vi "NR do Call Process.vi"(8 "error in (no error)":errorcluster caption="에러 입력(에러 없음)", 9 "Waiting Time":i32, 10 "Max Retry Count":i32, 11 "Instrument Manager 입력":refnum<class "Instrument Manager.lvclass">) -> (0 "error out":errorcluster caption="에러 출력", 2 "Connected?":bool, 3 "Instrument Manager 출력":refnum<class "Instrument Manager.lvclass">)   [LabVIEW 2023, in "Instrument Manager.lvclass"]
uses:
  Instrument Manager.lvclass
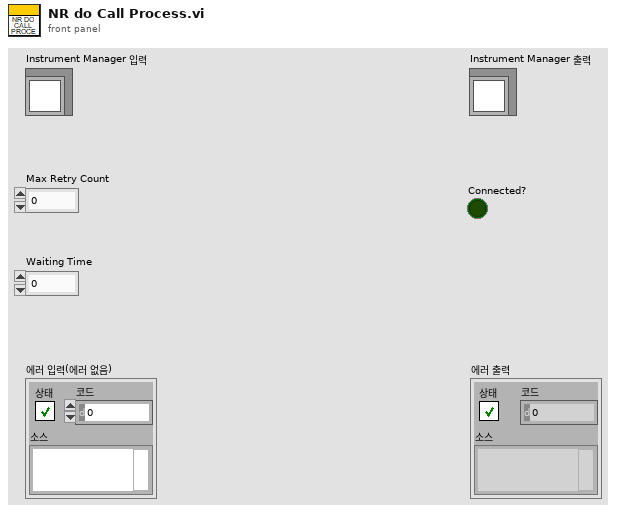
[diagram p1: front panel]
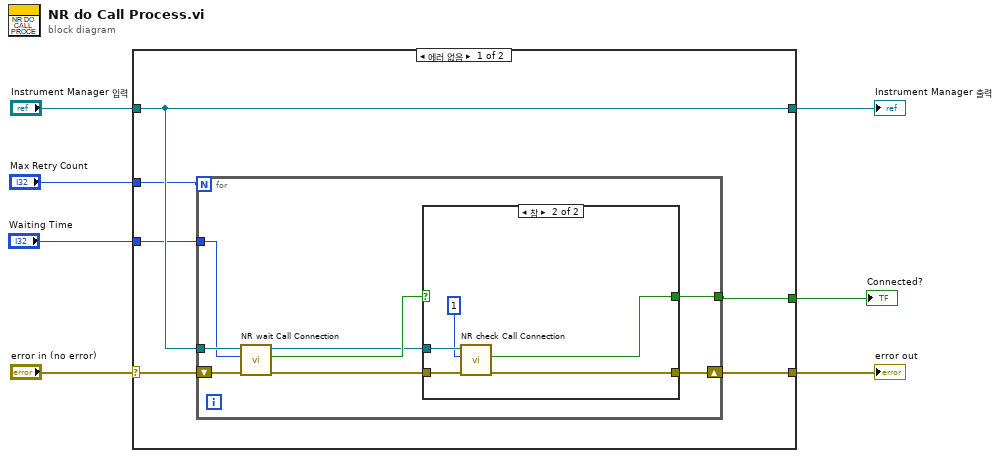
[diagram p0: block diagram]
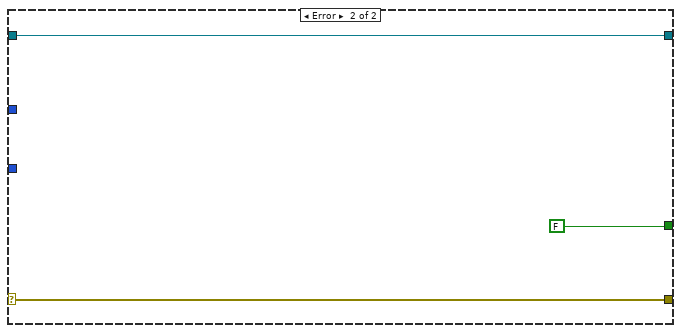
[diagram p3: hidden frame]
diagram:
  n1 = case shown="에러 없음" "error in (no error)" {
    selector: "error in (no error)" -> [w9 w31]
    tunnel: [w10 w31] -> w6
    tunnel: [w13 w30] -> w4
    tunnel: "Instrument Manager 입력" -> [w13 w30]
    tunnel: "Waiting Time" -> [w12 _]
    tunnel: "Max Retry Count" -> [w11 _]
    tunnel: [w8 FALSE ("Connected?")] -> w1
    frame No Error {
      n2 = for {
        N: w11 -> [_]
        tunnel: w13 -> [w21]
        tunnel: w12 -> [w20]
        tunnel: [w16] -> w8
        shift-right: [w15] -> w10
        shift-left: w9 -> [w14]
        n3 = call "NR wait Call Connection.vi"("error in (no error)"=w14, "Waiting Time"=w20, "Instrument Manager 입력"=w21) -> ("error out"=w17:errorcluster, "Connected?"=w19:bool, "Instrument Manager 출력"=w18:refnum<class "Instrument Manager.lvclass">)  [unwired: 6 in]
        n4 = case shown="참" w19 {
          selector: w19 -> [w23 _]
          tunnel: w18 -> [_ w28]
          tunnel: w17 -> [w22 w27]
          tunnel: [w23 w25] -> w16
          tunnel: [w22 w26] -> w15
          frame False {
          }
          frame True {
            n5 = call "NR check Call Connection.vi"("error in (no error)"=w27, "Waiting TIme"=1, "Instrument Manager 입력"=w28) -> ("error out"=w26:errorcluster, "Connected?"=w25:bool)  [unwired: 6 in, 1 out]
          }
        }
      }
    }
    frame Error {
    }
  }
  "error out" <- w6
  "Instrument Manager 출력" <- w4
  "Connected?" <- w1
